vi "VIH ProjFile - XML - Property Element - Read.vi"(8 "error in":errorcluster, 11 "XML Node":refnum<k20>) -> (0 "error out":errorcluster, 1 "Property Value":string, 2 "Property Name":string, 3 "dup XML Node":refnum<k20>)   [LabVIEW 2014]
doc: "::: VI Helpeks :::\nCopyright (c) 2000-2026 Konstantin Shifershteyn. All rights reserved."
uses:
  <vilib>/xml/Close Reference(Node).vi
  <vilib>/xml/Close Reference(NNMap).vi
  <resource>/objmgr/DOMUserDefRef.rc
  <vilib>/xml/NI_XML.lvlib
panel:
  # "VI Helpeks\nCopyright (c) 2012-2026 Konstantin Shifershteyn"
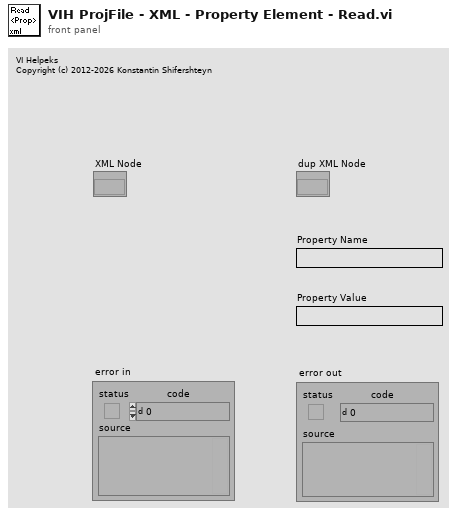
[diagram p1: front panel]
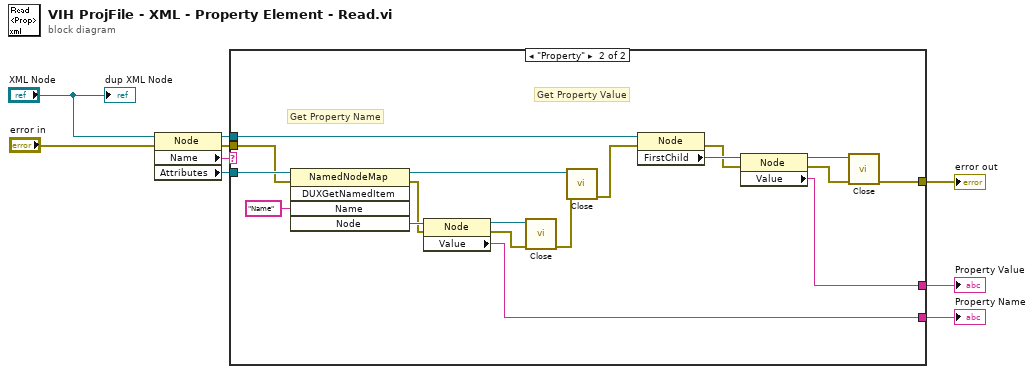
[diagram p0: block diagram]
diagram:
  n1 = property class="Node"(reference="XML Node", error in="error in") -> (reference out=w6:refnum<k20>, error out=w7:errorcluster, "Name"=w9:string, "Attributes"=w8:refnum<k20>)
  n2 = case shown="\"Property\"" w9 {
    tunnel: w8 -> [_ w26]
    tunnel: w7 -> [w10 w23]
    tunnel: [w10 w16] -> w1
    tunnel: w6 -> [_ w19]
    tunnel: [_ w11] -> w3
    tunnel: [_ w15] -> w2
    frame Default {
    }
    frame "Property" {
      # "Get Property Value"
      # "Get Property Name"
      n3 = invoke class="NamedNodeMap" method="DUXGetNamedItem"(reference=w26, error in=w23, "Name"="Name") -> (reference out=w24:refnum<k20>, error out=w22:errorcluster, "Node"=w28:refnum<k20>)  [unwired: 2 in, 2 out]
      n4 = property class="Node"(reference=w28, error in=w22) -> (reference out=w27:refnum<k20>, error out=w14:errorcluster, "Value"=w15:string)
      n5 = call-poly <vilib>:"Close.vi"("error in (no error)"=w14, "node"=w27) -> ("error out"=w17:errorcluster)  [unwired: 7 in]
      n6 = call-poly <vilib>:"Close.vi"("error in (no error)"=w17, "named node map"=w24) -> ("error out"=w13:errorcluster)  [unwired: 7 in]
      n7 = property class="Node"(reference=w19, error in=w13) -> (error out=w20:errorcluster, "FirstChild"=w21:refnum<k20>)  [unwired: 1 out]
      n8 = property class="Node"(reference=w21, error in=w20) -> (reference out=w18:refnum<k20>, error out=w12:errorcluster, "Value"=w11:string)
      n9 = call-poly <vilib>:"Close.vi"("error in (no error)"=w12, "node"=w18) -> ("error out"=w16:errorcluster)  [unwired: 7 in]
    }
  }
  "error out" <- w1
  "Property Name" <- w2
  "Property Value" <- w3
  "dup XML Node" <- "XML Node"
